vi "Express VI - Filter ECG.vi"() -> ()   [LabVIEW 2020]
doc: "This example shows some results of the use of the Filter Express VI."
uses:
  <vilib>/express/express analysis/Spectral/Block/exnSpectralBlock spectral measurements PSD poly.vi
  <vilib>/express/express analysis/Spectral/Block/exnSpectralBlock spectral measurements PSD WFM.vi
  <vilib>/express/express analysis/Spectral/XNode/ExpressSpectralMeasurementsBlockNode.xnode
  <vilib>/measure/NI_MABase.lvlib
panel:
  out "PSD 2":cluster{"f0":dbl, "df":dbl, "magnitude":dbl[]}(graph)
  in  "Simulation Mode":enum16{"Baseline", "No Baseline"}(ring)
  out "Sine waveform":waveform(dbl)(graph)
  in  "fc":dbl=50.0 caption="Lower Cut-Off"
  in  "fc":dbl=100.0 caption="Lower Cut-Off"
  out "PSD":cluster{"f0":dbl, "df":dbl, "magnitude":dbl[]}(graph)
  out "Highpass Results":dynamicdata(graph)
  out "Lowpass Results":dynamicdata(graph)
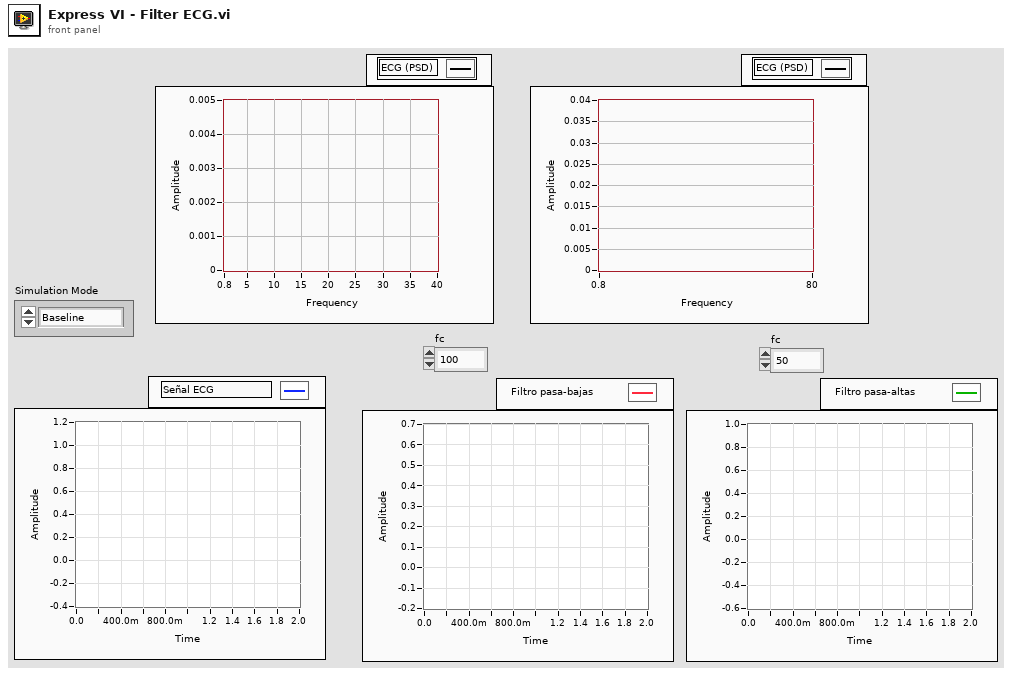
[diagram p1: front panel]
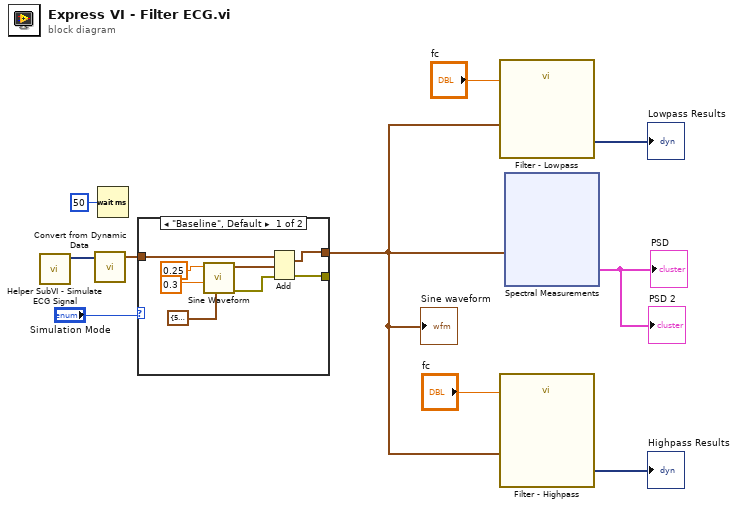
[diagram p0: block diagram]
diagram:
  n1 = call "Helper SubVI - Simulate ECG Signal.vi"() -> ("Data"=w5:dynamicdata)  [unwired: 11 in]
  n2 = call "Convert from Dynamic Data"("Dynamic Data Type"=w5) -> ("Waveform"=w4:waveform(dbl))  [unwired: 1 in, 2 out]
  n3 = Wait (ms)(milliseconds to wait=u32 50 ("millisecond multiple")) -> ()  [unwired: 1 out]
  n4 = case shown="\"Baseline\", Default" "Simulation Mode" {
    tunnel: w4 -> [w15 w19]
    tunnel: [w13 w19] -> w2
    tunnel: [w11 _] -> _
    frame "Baseline", Default {
      n5 = call <vilib>:"Sine Waveform.vi"("sampling info"=cluster{"Fs":dbl, "#s":dbl} {"Fs"=500.0, "#s"=500.0}, "amplitude"=0.3, "frequency"=0.25) -> ("error out"=w12:errorcluster, "signal out"=w14:waveform(dbl))  [unwired: 4 in, 3 out]
      n6 = Add(1:w14, 2:w15, 4:w12) -> (0:w13:waveform(dbl), 3:w11:errorcluster)
    }
    frame "No Baseline" {
    }
  }
  "Sine waveform" <- w2
  n7 = call "Filter - Lowpass"("Lower Cut-Off"="fc", "Signal"=w2) -> ("Filtered Signal"=→"Lowpass Results":dynamicdata)  [unwired: 8 in, 1 out]
  n8 = call "Filter - Highpass"("Lower Cut-Off"="fc", "Signal"=w2) -> ("Filtered Signal"=→"Highpass Results":dynamicdata)  [unwired: 8 in, 1 out]
  n9 = xnode "Spectral Measurements"("Signals"=w2) -> ("PSD"=→"PSD" →"PSD 2":cluster{"f0":dbl, "df":dbl, "magnitude":dbl[]})  [unwired: 1 in, 1 out]
